vi "1_Sin(x)_Cos(x)(Training).vi"() -> ()   [LabVIEW 2020]
uses:
  <vilib>/Ngene/Deep Learning Toolkit/Toolkit/NN_Train/Controls/NN_Train_Params.ctl
  <vilib>/Ngene/Deep Learning Toolkit/Toolkit/NN_Train/Controls/NN_Train_Optimizer.ctl
  <vilib>/Ngene/Deep Learning Toolkit/Toolkit/NN_Train/Controls/NN_Train_Data_Sampling.ctl
  <vilib>/Ngene/Deep Learning Toolkit/Toolkit/NN_Train/Controls/NN_LR_Policy_Cfg.ctl
  <vilib>/Ngene/Deep Learning Toolkit/Toolkit/NN_Train/Controls/NN_LR_Policy_Type.ctl
  <vilib>/Ngene/Deep Learning Toolkit/Toolkit/NN_Train/Controls/NN_Train_Session_Data.ctl
  <vilib>/Ngene/Deep Learning Toolkit/Toolkit/NN_Layers/Layers/FC/Controls/NN_Layer_Config(FC).ctl
  <vilib>/Ngene/Deep Learning Toolkit/Toolkit/NN_Layers/Layers/BatchNorm/Controls/NN_BN_Params.ctl
  <vilib>/Ngene/Deep Learning Toolkit/Toolkit/NN_Activations/Controls/NN_Activation_Type.ctl
  <vilib>/Ngene/Deep Learning Toolkit/Toolkit/NN_Layers/Controls/NN_Layer_Init_Params.ctl
  <vilib>/Ngene/Deep Learning Toolkit/Toolkit/NN_Layers/Controls/NN_Layer_Weight_Init_Type.ctl
  <vilib>/Ngene/Deep Learning Toolkit/Toolkit/NN_Network/Controls/NN_Save_Before_Destroy_Options.ctl
  <vilib>/Ngene/Deep Learning Toolkit/Toolkit/NN_Network/Controls/NN_Device.ctl
  <vilib>/Ngene/Deep Learning Toolkit/Toolkit/NN_Layers/Layers/Input/Controls/NN_Layer_Config(Input1D).ctl
  <vilib>/Ngene/Deep Learning Toolkit/Toolkit/NN_Data/Controls/NN_Data_type.ctl
  <vilib>/Ngene/Deep Learning Toolkit/Toolkit/NN_Data/API/DataSet/DataSet_Types/NN_DataSet(In1D_Out1D).ctl
  <vilib>/Ngene/Deep Learning Toolkit/Toolkit/NN_Data/Controls/DataRef_Types/2D/NN_Data_ref(2D_SGL).ctl
  <vilib>/Analysis/1siggen.llb/Ramp Pattern by Samples.vi
  <vilib>/Ngene/Deep Learning Toolkit/Toolkit/NN_Layers/Layers/Input/NN_Layer_Create(Input1D).vi
  <vilib>/Ngene/Deep Learning Toolkit/Toolkit/NN_Layers/Layers/FC/NN_Layer_Create(FC).vi
  <vilib>/Ngene/Deep Learning Toolkit/Toolkit/NN_Train/Loss_Functions/NN_Set_Loss(MSE).vi
  <vilib>/Ngene/Deep Learning Toolkit/Toolkit/NN_Train/SubVIs/Dataset_Checks/NN_Check_Dataset(In1D_Out1D).vi
  <vilib>/Ngene/Deep Learning Toolkit/Toolkit/NN_Data/subVIs/Get_Data_Vals/2D/NN_Data_Get_ValByRef(2D_SGL).vi
  <vilib>/Ngene/Deep Learning Toolkit/Toolkit/NN_Network/subVIs/NN_Predict/NN_Predict(In1D_Out1D).vi
  <vilib>/Ngene/Deep Learning Toolkit/Toolkit/NN_Train/Eval_Loss/NN_Eval_Test_Error_Loss/NN_Eval(In1D_Out1D).vi
  <vilib>/Ngene/Deep Learning Toolkit/Toolkit/Deep_Learning_Toolkit_by_Ngene.lvlib
  <vilib>/Analysis/NI_AALBase.lvlib
panel:
  out "Cos(x): Predictions vs Ground Truths":sgl[][](graph)
  out "Loop Time":dbl=0.043440699999337085 format="%#_4p"
  out "Test Loss":sgl=0.00088836974
  out "Training Loss":sgl=0.00065941934
  in  "Stop":bool
  out "Loss Graphs":cluster{"Loss":sgl, "Test Loss":sgl}(graph)={"Loss"=0.00065941934, "Test Loss"=0.0007708679}
  in  "# of Sine Cycles":dbl=5.0
  out "Sin(x): Predictions vs Ground Truths":sgl[][](graph)
  in  "Eval?":bool
  out "Session Data":T1={"Epochs"=464.512, "Tot_Iter"=7258, "LR"=0.0025, "LR_iter"=7259}
  in  "LR_Decay_Params":T2={"Policy_Type"=enum."Step", "LR0"=0.01, "k"=200.0, "WarmUp_Policy"=enum."Ramp", "WarmUp_Iter"=100, "WarmUp_Ratio"=10.0} {"WarmUp_Ratio" min=1; "WarmUp_Iter" min=1; "LR0" format="%.7f"}
  in  "NN_Train_Params":T4={"Optimizer"=enum."Adam", "Beta_1"=0.9, "Beta_2"=0.999, "Weight Decay(L1)"=1e-08, "Weight Decay(L2)"=1e-08, "Data_Sampling"=enum."Random"}
  # "Overview: Demonstrates the usage of DeepLTK (Deep Learning Toolkit for LabVIEW) for solving a simple regression problem of modeling sin(x) and cos(x) function.\nRequirements: DeepLTK - Deep Learning Toolkit for LabVIEW (https://www.ngene.co/deep-learning-toolkit-for-labview)\nInstructions:\n1. Run the VI with default configurations.\n2. Observe how the training loss is decreasing.\n3. Periodically press \"Eval?\" button to observe \"Test Loss\" and performance of the model on Test Dataset\n4. Press \"Stop\" when \"Test Loss\" is is not decreasing. ~500 epochs\nMore Examples:  https://github.com/ngenehub/deepltk_examples"
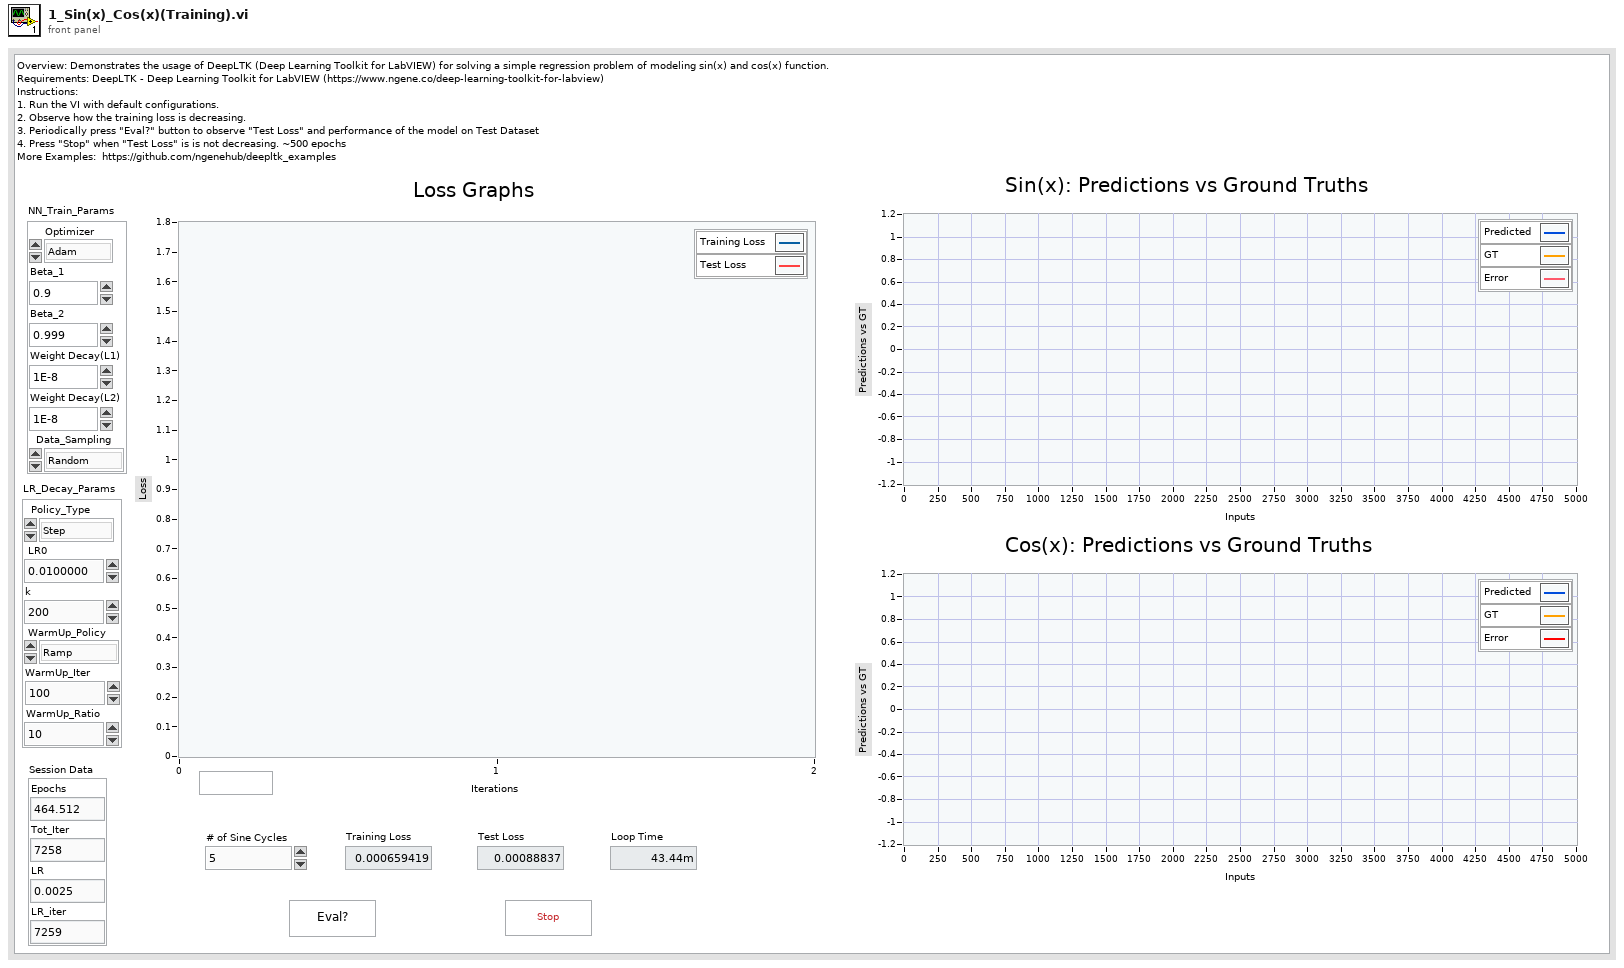
[diagram p1: front panel]
types:
  T1 = typedef "Deep_Learning_Toolkit_by_Ngene.lvlib/NN_Train_Session_Data.ctl" = cluster{"Epochs":sgl, "Tot_Iter":i32, "LR":sgl, "LR_iter":i32}
  T2 = typedef "Deep_Learning_Toolkit_by_Ngene.lvlib/NN_LR_Policy_Cfg.ctl" = cluster{"Policy_Type":T3, "LR0":dbl, "k":sgl, "WarmUp_Policy":enum16{"Step", "Ramp"}, "WarmUp_Iter":i32, "WarmUp_Ratio":sgl}
  T3 = typedef "Deep_Learning_Toolkit_by_Ngene.lvlib/NN_LR_Policy_Type.ctl" = enum16{"Manual", "Step", "Exp", "1/t"}
  T4 = typedef "Deep_Learning_Toolkit_by_Ngene.lvlib/NN_Train_Params.ctl" = cluster{"Optimizer":T5, "Beta_1":sgl, "Beta_2":sgl, "Weight Decay(L1)":sgl, "Weight Decay(L2)":sgl, "Data_Sampling":T6}
  T5 = typedef "Deep_Learning_Toolkit_by_Ngene.lvlib/NN_Train_Optimizer.ctl" = enum16{"SGD", "Adam", "Adagrad", "Adadelta", "RMSProp", "Nesterov"}
  T6 = typedef "Deep_Learning_Toolkit_by_Ngene.lvlib/NN_Train_Data_Sampling.ctl" = enum16{"Random", "Sequential"}
  T7 = typedef "Deep_Learning_Toolkit_by_Ngene.lvlib/NN_DataSet(In1D_Out1D).ctl" = cluster{"Inputs Ref.":variant, "Outputs Ref.":T8, "Dims_In":i32, "Dataset_Size":i32, "Dims_Out":i32, "Labels":string[], "File Paths":path[], "Custom_Data":variant}
  T8 = typedef "Deep_Learning_Toolkit_by_Ngene.lvlib/NN_Data_ref(2D_SGL).ctl" = refnum<data-value>
  T9 = typedef "Deep_Learning_Toolkit_by_Ngene.lvlib/NN_Layer_Config(Input1D).ctl" = cluster{"Name":string, "Size":i32, "Data_Type":T10, "Shift":sgl, "Scale":sgl}
  T10 = typedef "Deep_Learning_Toolkit_by_Ngene.lvlib/NN_Data_type.ctl" = enum16{"I8", "U8", "I16", "U16", "U32 ARGB", "SGL"}
  T11 = typedef "Deep_Learning_Toolkit_by_Ngene.lvlib/NN_Device.ctl" = enum16{"CPU", "GPU"}
  T12 = typedef "Deep_Learning_Toolkit_by_Ngene.lvlib/NN_Save_Before_Destroy_Options.ctl" = cluster{"CFG?":bool, "Weights?":bool, "Render?":bool}
  T13 = typedef "Deep_Learning_Toolkit_by_Ngene.lvlib/NN_Layer_Config(FC).ctl" = cluster{"Name":string, "Size":i32, "BN":bool, "BN_Params":T14, "Activation":T15, "Has Bias?":bool, "Init_Params":T16, "Custom_Params":string}
  T14 = typedef "Deep_Learning_Toolkit_by_Ngene.lvlib/NN_BN_Params.ctl" = cluster{"epsilon":sgl, "momentum":sgl}
  T15 = typedef "Deep_Learning_Toolkit_by_Ngene.lvlib/NN_Activation_Type.ctl" = enum16{"Sigmoid", "ReLU", "LReLU", "ReLU6", "GELU", "tanh", "Swish", "Mish", "None"}
  T16 = typedef "Deep_Learning_Toolkit_by_Ngene.lvlib/NN_Layer_Init_Params.ctl" = cluster{"Init_Type":T17, "Value":sgl}
  T17 = typedef "Deep_Learning_Toolkit_by_Ngene.lvlib/NN_Layer_Weight_Init_Type.ctl" = enum16{"Const", "Uniform", "Gaussian", "Xavier"}
  T18 = typedef "Deep_Learning_Toolkit_by_Ngene.lvlib/NN.ctl" = cluster{"Name":string, "No of Layers":i32, "mBatch":i32, "Layers":T19[], "Dimty":T20, "Dims_In":T21, "Dims_Out":T21, "Working_Dir":path, "Train?":bool, "Train_Params":T4, "LR_Update_Policy":T2, "Session Data":T1, "Ground_truth":T22, "NNg_hdls":T23, "NN_Device":T11, "GPU Id":i32, "Labels":string[], "Loss_Type":T24, "Loss_Cfg_Prms":variant, "NNG_WS":T25, "DryRun?":bool}
  T19 = typedef "Deep_Learning_Toolkit_by_Ngene.lvlib/NN_Layer_ref.ctl" = refnum<file>
  T20 = typedef "Deep_Learning_Toolkit_by_Ngene.lvlib/NN_In_Out_Dim-ty.ctl" = enum8{"In1D_Out1D", "In3D_Out1D", "In3D_Out3D", "In3D_OutBBox"}
  T21 = typedef "Deep_Learning_Toolkit_by_Ngene.lvlib/NN_Dims(C,H,W).ctl" = cluster{"C":i32, "H":i32, "W":i32}
  T22 = typedef "Deep_Learning_Toolkit_by_Ngene.lvlib/NN_Ground_truth.ctl" = cluster{"Y":variant}
  T23 = typedef "Deep_Learning_Toolkit_by_Ngene.lvlib/nng_cuda_handles.ctl" = cluster{"cudnn":u64, "cublas":u64, "stream":u64, "curand":u64}
  T24 = typedef "Deep_Learning_Toolkit_by_Ngene.lvlib/NN_Loss_Type.ctl" = enum16{"None", "MSE", "CrossEntropy", "YOLO_v2", "YOLO_v4"}
  T25 = typedef "Deep_Learning_Toolkit_by_Ngene.lvlib/NNG_WS.ctl" = cluster{"NNG_WS_Mem":T26, "Max_WS_Size":i64}
  T26 = typedef "Deep_Learning_Toolkit_by_Ngene.lvlib/NNg_WS_Mem_DVR.ctl" = refnum<data-value>
  T27 = typedef "Deep_Learning_Toolkit_by_Ngene.lvlib/NN_Eval_Params.ctl" = cluster{"Loss":sgl, "Error":sgl}
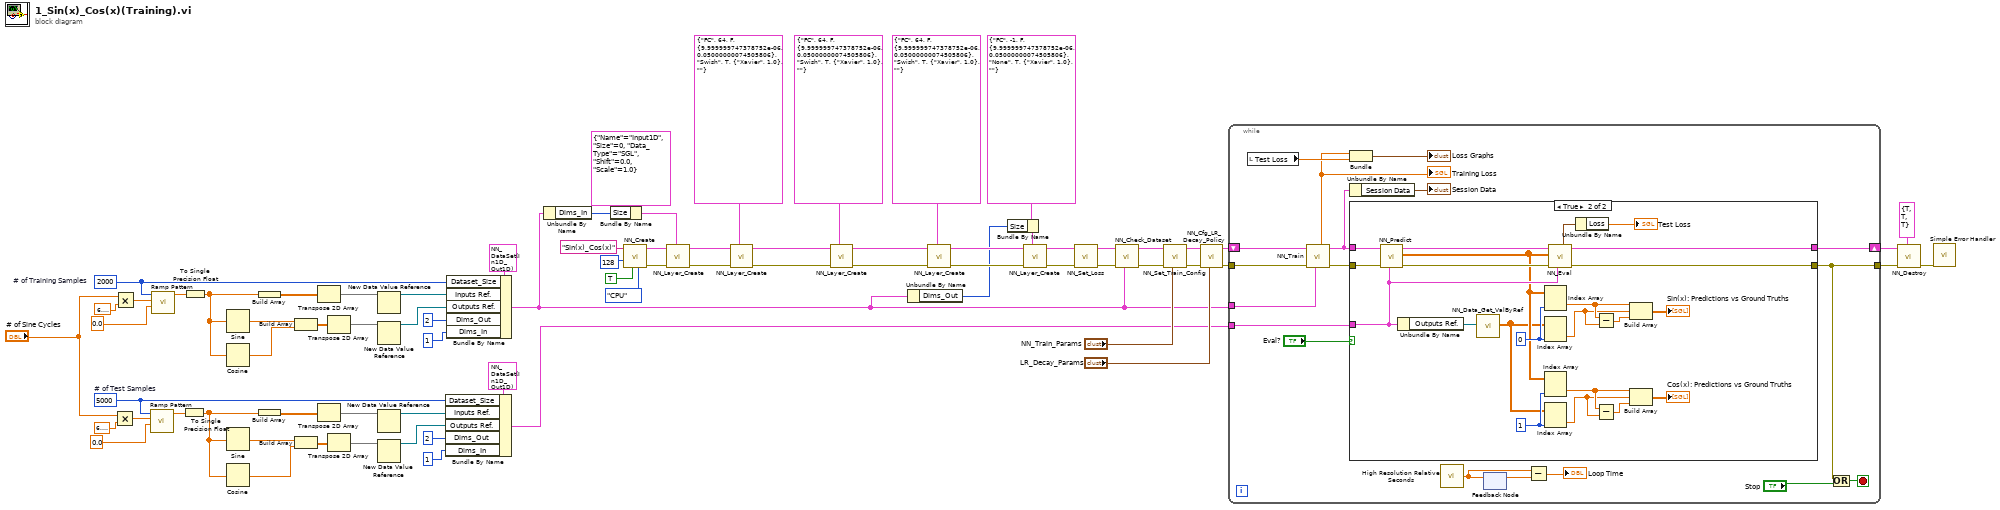
[diagram p0: block diagram]
diagram:
  w67 = 2000  # # of Training Samples
  w72 = 5000  # # of Test Samples
  n1 = Multiply(x="# of Sine Cycles", y=6.283185307179586) -> (x*y=w75:dbl)
  n2 = Multiply(x="# of Sine Cycles", y=6.283185307179586) -> (x*y=w70:dbl)
  n3 = call-poly <vilib>:"Ramp Pattern.vi"("start"=0.0, "end"=w75, "samples"=w72) -> ("Ramp Pattern"=w74:dbl[])  [unwired: 7 in, 1 out]
  n4 = call-poly <vilib>:"Ramp Pattern.vi"("start"=0.0, "end"=w70, "samples"=w67) -> ("Ramp Pattern"=w69:dbl[])  [unwired: 7 in, 1 out]
  n5 = To Single Precision Float(number=w74) -> (single precision float=w65:sgl[])
  n6 = To Single Precision Float(number=w69) -> (single precision float=w58:sgl[])
  n7 = Sine(x=w58) -> (sin(x)=w60:sgl[])
  n8 = Cosine(x=w58) -> (cos(x)=w59:sgl[])
  n9 = Sine(x=w65) -> (sin(x)=w62:sgl[])
  n10 = Cosine(x=w65) -> (cos(x)=w63:sgl[])
  n11 = Build Array(w58) -> (w54:sgl[][])
  n12 = Build Array(w65) -> (w56:sgl[][])
  n13 = Build Array(w60, w59) -> (w61:sgl[][])
  n14 = Build Array(w62, w63) -> (w64:sgl[][])
  n15 = Transpose 2D Array(2D array=w54) -> (transposed array=w3:sgl[][])
  n16 = Transpose 2D Array(2D array=w56) -> (transposed array=w2:sgl[][])
  n17 = Transpose 2D Array(2D array=w61) -> (transposed array=w57:sgl[][])
  n18 = Transpose 2D Array(2D array=w64) -> (transposed array=w55:sgl[][])
  n19 = New Data Value Reference(data value=w2) -> (data value reference=w22:refnum<data-value>)  [unwired: 1 in, 1 out]
  n20 = New Data Value Reference(data value=w55) -> (data value reference=w21:refnum<data-value>)  [unwired: 1 in, 1 out]
  n21 = New Data Value Reference(data value=w3) -> (data value reference=w18:refnum<data-value>)  [unwired: 1 in, 1 out]
  n22 = New Data Value Reference(data value=w57) -> (data value reference=w17:refnum<data-value>)  [unwired: 1 in, 1 out]
  n23 = Bundle By Name(cluster=T7 {"Inputs Ref."=variant(refnum<data-value> refnum), "Outputs Ref."=refnum, "Dims_In"=0, "Dataset_Size"=0, "Dims_Out"=0, "Labels"=[], "File Paths"=[], "Custom_Data"=variant} ("Dataset(In1D_Out1D)"), "Dataset_Size"=w72, "Inputs Ref."=w22, "Outputs Ref."=w21, "Dims_Out"=2, "Dims_In"=1 ("Dims_Out")) -> (w20:T7)
  n24 = Bundle By Name(cluster=T7 {"Inputs Ref."=variant(refnum<data-value> refnum), "Outputs Ref."=refnum, "Dims_In"=0, "Dataset_Size"=0, "Dims_Out"=0, "Labels"=[], "File Paths"=[], "Custom_Data"=variant} ("Dataset(In1D_Out1D)"), "Dataset_Size"=w67, "Inputs Ref."=w18, "Outputs Ref."=w17, "Dims_Out"=2, "Dims_In"=1 ("Dims_Out")) -> (w7:T7)
  n25 = Unbundle By Name(w7) -> ("Dims_In"=w27:i32)
  n26 = Bundle By Name(cluster=T9 {"Name"="Input1D", "Size"=0, "Data_Type"=enum."SGL", "Shift"=0.0, "Scale"=1.0} ("Input1D_Cfg"), "Size"=w27) -> (w45:T9)
  n27 = call <vilib>:"NN_Create.vi"("NN_Device"=NN_Device."CPU", "Train? (false)"=TRUE, "mBatch (1)"=128, "Name"="Sin(x)_Cos(x)") -> ("error out"=w50:errorcluster, "NN out"=w51:T18)  [unwired: 6 in]
  n28 = call-poly <vilib>:"NN_Layer_Create.vi"("Input1D_Cfg"=w45, "error in (no error)"=w50, "NN in"=w51) -> ("error out"=w53:errorcluster, "NN out"=w52:T18)  [unwired: 6 in, 1 out]
  n29 = call-poly <vilib>:"NN_Layer_Create.vi"("FC_Cfg"=T13 {"Name"="FC", "Size"=64, "BN"=FALSE, "BN_Params"={"epsilon"=1e-05, "momentum"=0.05}, "Activation"=enum."Swish", "Has Bias?"=TRUE, "Init_Params"={"Init_Type"=enum."Xavier", "Value"=1.0}, "Custom_Params"=""}, "error in (no error)"=w53, "NN in"=w52) -> ("error out"=w25:errorcluster, "NN out"=w26:T18)  [unwired: 6 in, 1 out]
  n30 = call-poly <vilib>:"NN_Layer_Create.vi"("FC_Cfg"=T13 {"Name"="FC", "Size"=64, "BN"=FALSE, "BN_Params"={"epsilon"=1e-05, "momentum"=0.05}, "Activation"=enum."Swish", "Has Bias?"=TRUE, "Init_Params"={"Init_Type"=enum."Xavier", "Value"=1.0}, "Custom_Params"=""}, "error in (no error)"=w25, "NN in"=w26) -> ("error out"=w13:errorcluster, "NN out"=w14:T18)  [unwired: 6 in, 1 out]
  n31 = Unbundle By Name(w7) -> ("Dims_Out"=w6:i32)
  n32 = call-poly <vilib>:"NN_Layer_Create.vi"("FC_Cfg"=T13 {"Name"="FC", "Size"=64, "BN"=FALSE, "BN_Params"={"epsilon"=1e-05, "momentum"=0.05}, "Activation"=enum."Swish", "Has Bias?"=TRUE, "Init_Params"={"Init_Type"=enum."Xavier", "Value"=1.0}, "Custom_Params"=""}, "error in (no error)"=w13, "NN in"=w14) -> ("error out"=w11:errorcluster, "NN out"=w12:T18)  [unwired: 6 in, 1 out]
  n33 = Bundle By Name(cluster=T13 {"Name"="FC", "Size"=-1, "BN"=FALSE, "BN_Params"={"epsilon"=1e-05, "momentum"=0.05}, "Activation"=enum."None", "Has Bias?"=TRUE, "Init_Params"={"Init_Type"=enum."Xavier", "Value"=1.0}, "Custom_Params"=""} ("FC_Cfg"), "Size"=w6) -> (w4:T13)
  n34 = call-poly <vilib>:"NN_Layer_Create.vi"("FC_Cfg"=w4, "error in (no error)"=w11, "NN in"=w12) -> ("error out"=w29:errorcluster, "NN out"=w28:T18)  [unwired: 6 in, 1 out]
  n35 = call-poly <vilib>:"NN_Set_Loss.vi"("error in (no error)"=w29, "NN in"=w28) -> ("error out"=w31:errorcluster, "NN out"=w43:T18)  [unwired: 8 in]
  n36 = call-poly <vilib>:"NN_Check_Dataset.vi"("Dataset"=w7, "error in (no error)"=w31, "NN in"=w43) -> ("error out"=w30:errorcluster, "NN out"=w32:T18)  [unwired: 7 in]
  n37 = call <vilib>:"NN_Set_Train_Config.vi"("NN_Train_Params"="NN_Train_Params", "error in (no error)"=w30, "NN in"=w32) -> ("error out"=w37:errorcluster, "NN out"=w42:T18)  [unwired: 7 in]
  n38 = call <vilib>:"NN_Cfg_LR_Decay_Policy.vi"("LR_Decay_Params"="LR_Decay_Params", "error in (no error)"=w37, "NN in"=w42) -> ("error out"=w36:errorcluster, "NN out"=w38:T18)  [unwired: 7 in]
  n39 = while {
    tunnel: w36 -> [w93]
    tunnel: w7 -> [w85]
    shift-right: [w89] -> w40
    shift-left: w38 -> [w94]
    tunnel: [w84] -> w39
    tunnel: w20 -> [w83]
    stop <- w92 stop-if-true
    n40 = local read "Test Loss"() -> (w86:sgl)
    n41 = call <vilib>:"NN_Train.vi"("Train Dataset"=w85, "error in (no error)"=w93, "NN in"=w94) -> ("error out"=w88:errorcluster, "NN out"=w91:T18, "Loss"=w77:sgl)  [unwired: 3 in, 3 out]
    "Training Loss" <- w77
    n42 = Bundle("Loss"=w77, "Test Loss"=w86) -> (→"Loss Graphs":cluster{"Loss":sgl, "Test Loss":sgl})  [unwired: 1 in]
    n43 = Unbundle By Name(w91) -> ("Session Data"=→"Session Data":T1)
    n44 = case shown="True" "Eval?" {
      tunnel: w91 -> [w96 w114]
      tunnel: [w96 w118] -> w89
      tunnel: w88 -> [w95 w113]
      tunnel: [w95 w117] -> w84
      tunnel: w83 -> [_ w112]
      frame False {
      }
      frame True {
        w109 = 1 ("disabled index (col)")
        w110 = 0 ("disabled index (col)")
        n45 = call-poly <vilib>:"NN_Predict.vi"("Dataset"=w112, "error in (no error)"=w113, "NN in"=w114) -> ("error out"=w115:errorcluster, "Predictions"=w108:sgl[][], "NN out"=w116:T18)  [unwired: 6 in]
        n46 = Unbundle By Name(w112) -> ("Outputs Ref."=w111:T8)
        n47 = call-poly <vilib>:"NN_Data_Get_ValByRef.vi"("DVR(2D_SGL)"=w111) -> ("Value(2D_SGL)"=w107:sgl[][])  [unwired: 7 in, 1 out]
        n48 = Index Array(array=w108, index (col)=w110) -> (element=w104:sgl[])  [unwired: 1 in]
        n49 = Index Array(array=w107, index (col)=w110) -> (element=w102:sgl[])  [unwired: 1 in]
        n50 = Index Array(array=w108, index (col)=w109) -> (element=w100:sgl[])  [unwired: 1 in]
        n51 = Index Array(array=w107, index (col)=w109) -> (element=w99:sgl[])  [unwired: 1 in]
        n52 = call-poly <vilib>:"NN_Eval.vi"("Dataset"=w112, "error in (no error)"=w115, "Predictions"=w108, "NN in"=w116) -> ("error out"=w117:errorcluster, "NN out"=w118:T18, "NN_Eval_Params"=w98:T27)  [unwired: 4 in, 1 out]
        n53 = Unbundle By Name(w98) -> ("Loss"=→"Test Loss":sgl)
        n54 = Subtract(x=w104, y=w102) -> (x-y=w103:sgl[])
        n55 = Subtract(x=w100, y=w99) -> (x-y=w101:sgl[])
        n56 = Build Array(w104, w102, w103) -> (→"Sin(x): Predictions vs Ground Truths":sgl[][])
        n57 = Build Array(w100, w99, w101) -> (→"Cos(x): Predictions vs Ground Truths":sgl[][])
      }
    }
    n58 = call <vilib>:"High Resolution Relative Seconds.vi"() -> ("relative seconds"=w82:dbl)
    n59 = feedback-in #1(w82) -> ()
    n60 = feedback #1() -> (w81:dbl)  [unwired: 1 in]
    n61 = Subtract(x=w82, y=w81) -> (x-y=→"Loop Time":dbl)
    n62 = Or(x=w84, y="Stop") -> (x .or. y?=w92:bool)
  }
  n63 = call <vilib>:"NN_Destroy.vi"("Save (T, T, T)"=T12 {"CFG?"=TRUE, "Weights?"=TRUE, "Render?"=TRUE}, "error in (no error)"=w39, "NN in"=w40) -> ("error out"=w1:errorcluster)  [unwired: 7 in, 1 out]
  n64 = call <vilib>:"Simple Error Handler.vi"("error in (no error)"=w1) -> ()  [unwired: 4 in, 5 out]
